vi "Build Message with Arguments++.vi"   [LabVIEW 2017, in "Communicable State Machine.lvlib"]
doc: "Builds CSM message strings and operation strings.\n\n\n> [!NOTE] <b>Message Building API</b>\n>\n> This type of API is only used to concatenate message strings and does not send messages directly. The strings need to be merged into the CSM state queue, and the messages will be sent and the operation executed within the Parse State Queue++ VI. If you are familiar with CSM rules, you do not need to use this type of API. You can type the corresponding message string or operation string directly into the string.\n\n\n> [!NOTE] <b>Polymorphic VI Options</b>\n> - Build Message with Arguments(Auto Check).vi: Concatenates message strings based on the input message symbols.\n> - Build Asynchronous Message with Arguments.vi: Concatenates and generates CSM asynchronous message strings. The message type symbol is `->`.\n> - Build No-Reply Asynchronous Message with Arguments.vi: Concatenates and generates CSM asynchronous message strings without reply. The message type symbol is `->|`.\n> - Build Synchronous Message with Arguments.vi: Concatenates and generates CSM synchronous message strings. The message type symbol is `-@`.\n> - Build Interrupt Broadcast Message.vi: Concatenates and generates CSM interrupt broadcast strings.\n> - Build Normal Broadcast Message.vi: Concatenates and generates CSM status broadcast strings.\n> - Build Register Message.vi: Concatenates and generates CSM register state operation strings.\n> - Build Unregister Message.vi: Concatenates and generates CSM unregister state operation strings.\n> - CSM - Replace Marks in Messages.vi: Replaces placeholders in message strings.\n> - CSM - Replace Mark with String Array.vi: Replaces tags in a single state string with strings from an array and merges them into a string describing a group of states.\n\n\n> [!NOTE] <b>CSM Inter-module Communication Types</b>\n>\n> Communication between CSM modules is divided into two categories: Messages and Broadcasts.\n> - <b>Messages</b>: 1:1 communication between modules. Based on the message handling method, it can be further divided into Synchronous Call (`-@`), Asynchronous Call (`->`), and Asynchronous Call without Reply (`->|`).\n> - <b>Broadcasts</b>: 1:N communication between modules. The broadcasting module pushes the broadcast to all modules registered to that broadcast. Based on the broadcast processing priority, it can be further divided into Status Broadcast and Interrupt Broadcast.\n\n\n### Build Message with Arguments(Auto Check).vi\nConcatenates and generates CSM message strings. The message type symbol is automatically detected based on the input <b>State with Arguments</b>.\n\n\n> [!NOTE] <b>Message Building API</b>\n>\n> This type of API is only used to concatenate message strings and does not send messages directly. The strings need to be merged into the CSM state queue, and the messages will be sent and the operation executed within the Parse State Queue++ VI. If you are familiar with CSM rules, you do not need to use this type of API. You can type the corresponding message string or operation string directly into the string.\n\n\n> [!NOTE] <b>CSM Message Target Module Description</b>\n>\n> In Normal Mode, the target module for a CSM message is the specified module name.\n> System-level modules start with a `.` in their name. The target module for a CSM message includes the `.` in the name. For example, if the requested module name is `.System`, the target module for the CSM message is `.System`.\n> In Worker Mode, the target module for a CSM message can only be the overall module name, not the node name. For example, if the requested module name is `Worker#`, the target module for the CSM message is `Worker`.\n> In Chain of Responsibility Mode, the target module for a CSM message can only be the overall module name, not the node name. For example, if the requested module name is `Chain$1`, the target module for the CSM message is `Chain`.\n\n\n-- <b>Controls</b> --\n- <b>State with Arguments</b>: CSM state string, which can contain arguments and target module information.\n- <b>Arguments (\"\")</b>: Argument information. Arguments contained in <b>State with Arguments</b> will be replaced.\n- <b>Target Module (\"\")</b>: Target module. If empty, the default module in <b>State with Arguments</b> will be used.\n\n-- <b>Indicators</b> --\n- <b>CSM Message String</b>: Concatenated CSM message string.\n\n### Build Synchronous Message with Arguments.vi\nConcatenates and generates CSM synchronous message strings. The message type symbol is `-@`, for example:\n\n Message >> Arguments -@ Target\n\n\n> [!NOTE] <b>Message Building API</b>\n>\n> This type of API is only used to concatenate message strings and does not send messages directly. The strings need to be merged into the CSM state queue, and the messages will be sent and the operation executed within the Parse State Queue++ VI. If you are familiar with CSM rules, you do not need to use this type of API. You can type the corresponding message string or operation string directly into the string.\n\n\n> [!NOTE] <b>Synchronous Message</b>\n>\n> A synchronous message is a type of message. After a CSM sends a synchronous message, it pauses state transitions and waits for the callee to complete message processing. Synchronous messages are described via `-@`. A call from one JKISM module to another via a synchronous message is called a synchronous call.\n>\n> <b>Errors occurring at the Caller</b>:\n> - If the input target module is `\"\"`, a `NO Target Error` is generated.\n> - If the input module does not exist, a `Target Error` is generated.\n> - If the input module exists but does not complete processing within the specified time, a `Timeout Error` is generated.\n>\n> <b>Caller waits for return</b>:\n> - If the caller is a CSM module, it stays in the Parse State the Queue++ VI.\n> - If it is an API call, it stays in the calling VI, such as the CSM - Send Message and Wait for Reply VI.\n>\n> <b>Return</b>:\n> - <b>If the caller is a CSM module</b>:\n> - Normally, it enters the `Response` state to handle the return.\n> - If an error occurs at the caller, it causes the CSM state machine to enter the `Error Handler` module to handle the error.\n> - If an error occurs at the callee, this information is still the result of the message. It is handled in the `Response` state and can be obtained from Additional Information.\n> - <b>If it is an API call</b>:\n> - The Response output is the return.\n> - Errors occurring at both the caller and callee are merged into the error cluster output.\n\n\n> [!NOTE] <b>CSM Message Target Module Description</b>\n>\n> In Normal Mode, the target module for a CSM message is the specified module name.\n> System-level modules start with a `.` in their name. The target module for a CSM message includes the `.` in the name. For example, if the requested module name is `.System`, the target module for the CSM message is `.System`.\n> In Worker Mode, the target module for a CSM message can only be the overall module name, not the node name. For example, if the requested module name is `Worker#`, the target module for the CSM message is `Worker`.\n> In Chain of Responsibility Mode, the target module for a CSM message can only be the overall module name, not the node name. For example, if the requested module name is `Chain$1`, the target module for the CSM message is `Chain`.\n\n\n-- <b>Controls</b> --\n- <b>State with Arguments</b>: CSM state string.\n- <b>Arguments (\"\")</b>: Argument information. Arguments contained in <b>State with Arguments</b> will be replaced.\n- <b>Target Module (\"\")</b>: Target module. If empty, the default module in <b>State with Arguments</b> will be used.\n\n-- <b>Indicators</b> --\n- <b>CSM Message String</b>: Concatenated CSM message string.\n\n### Build Asynchronous Message with Arguments.vi\nConcatenates and generates CSM asynchronous message strings. The message type symbol is `->`, for example:\n\n Message >> Arguments -> Target\n\n\n> [!NOTE] <b>Message Building API</b>\n>\n> This type of API is only used to concatenate message strings and does not send messages directly. The strings need to be merged into the CSM state queue, and the messages will be sent and the operation executed within the Parse State Queue++ VI. If you are familiar with CSM rules, you do not need to use this type of API. You can type the corresponding message string or operation string directly into the string.\n\n\n> [!NOTE] <b>Asynchronous Message</b>\n>\n> An asynchronous message is a type of message. After a CSM sends an asynchronous message, it immediately continues to execute subsequent code without waiting for the callee to complete message processing. Asynchronous messages are divided into Asynchronous Call (`->`) and Asynchronous Call without Reply (`->|`). The only difference is that with an Asynchronous Call without Reply (`->|`), the callee will not return the result to the caller after completing the operation.\n>\n> <b>Errors occurring at the Caller</b>:\n> - If the input target module is `\"\"`, a `NO Target Error` is generated.\n> - If the input module does not exist, a `Target Error` is generated.\n>\n> <b>Caller does not wait for return</b>:\n> - If the caller is a CSM module, it enters the `Async Message Posted` state after sending the message in the Parse State Queue++ VI.\n> - If it is an API call, it continues to execute subsequent code. The API can only send Asynchronous without Reply messages.\n>\n> <b>Return</b>:\n> - <b>If the caller is a CSM module</b>:\n> - Normally, it enters the `Async Response` state to handle the return. If an error occurs at the callee, this information is still the result of the message. It is handled in the `Async Response` state, and this error information can be obtained from Additional Information.\n> - If an error occurs at the caller, it causes the CSM state machine to enter the `Error Handler` module to handle the error.\n> - There is no return if the API can only send Asynchronous without Reply messages.\n\n\n> [!NOTE] <b>CSM Message Target Module Description</b>\n>\n> In Normal Mode, the target module for a CSM message is the specified module name.\n> System-level modules start with a `.` in their name. The target module for a CSM message includes the `.` in the name. For example, if the requested module name is `.System`, the target module for the CSM message is `.System`.\n> In Worker Mode, the target module for a CSM message can only be the overall module name, not the node name. For example, if the requested module name is `Worker#`, the target module for the CSM message is `Worker`.\n> In Chain of Responsibility Mode, the target module for a CSM message can only be the overall module name, not the node name. For example, if the requested module name is `Chain$1`, the target module for the CSM message is `Chain`.\n\n\n-- <b>Controls</b> --\n- <b>State with Arguments</b>: CSM state string.\n- <b>Arguments (\"\")</b>: Argument information. Arguments contained in <b>State with Arguments</b> will be replaced.\n- <b>Target Module (\"\")</b>: Target module. If empty, the default module in <b>State with Arguments</b> will be used.\n\n-- <b>Indicators</b> --\n- <b>CSM Message String</b>: Concatenated CSM message string.\n\n### Build No-Reply Asynchronous Message with Arguments.vi\nConcatenates and generates CSM asynchronous message strings without reply. The message type symbol is `->|`, for example:\n\n Message >> Arguments ->| Target\n\n\n> [!NOTE] <b>Message Building API</b>\n>\n> This type of API is only used to concatenate message strings and does not send messages directly. The strings need to be merged into the CSM state queue, and the messages will be sent and the operation executed within the Parse State Queue++ VI. If you are familiar with CSM rules, you do not need to use this type of API. You can type the corresponding message string or operation string directly into the string.\n\n\n> [!NOTE] <b>Asynchronous Message</b>\n>\n> An asynchronous message is a type of message. After a CSM sends an asynchronous message, it immediately continues to execute subsequent code without waiting for the callee to complete message processing. Asynchronous messages are divided into Asynchronous Call (`->`) and Asynchronous Call without Reply (`->|`). The only difference is that with an Asynchronous Call without Reply (`->|`), the callee will not return the result to the caller after completing the operation.\n>\n> <b>Errors occurring at the Caller</b>:\n> - If the input target module is `\"\"`, a `NO Target Error` is generated.\n> - If the input module does not exist, a `Target Error` is generated.\n>\n> <b>Caller does not wait for return</b>:\n> - If the caller is a CSM module, it enters the `Async Message Posted` state after sending the message in the Parse State Queue++ VI.\n> - If it is an API call, it continues to execute subsequent code. The API can only send Asynchronous without Reply messages.\n>\n> <b>Return</b>:\n> - <b>If the caller is a CSM module</b>:\n> - Normally, it enters the `Async Response` state to handle the return. If an error occurs at the callee, this information is still the result of the message. It is handled in the `Async Response` state, and this error information can be obtained from Additional Information.\n> - If an error occurs at the caller, it causes the CSM state machine to enter the `Error Handler` module to handle the error.\n> - There is no return if the API can only send Asynchronous without Reply messages.\n\n\n> [!NOTE] <b>CSM Message Target Module Description</b>\n>\n> In Normal Mode, the target module for a CSM message is the specified module name.\n> System-level modules start with a `.` in their name. The target module for a CSM message includes the `.` in the name. For example, if the requested module name is `.System`, the target module for the CSM message is `.System`.\n> In Worker Mode, the target module for a CSM message can only be the overall module name, not the node name. For example, if the requested module name is `Worker#`, the target module for the CSM message is `Worker`.\n> In Chain of Responsibility Mode, the target module for a CSM message can only be the overall module name, not the node name. For example, if the requested module name is `Chain$1`, the target module for the CSM message is `Chain`.\n\n\n-- <b>Controls</b> --\n- <b>State with Arguments</b>: CSM state string.\n- <b>Arguments (\"\")</b>: Argument information. Arguments contained in <b>State with Arguments</b> will be replaced.\n- <b>Target Module (\"\")</b>: Target module. If empty, the default module in <b>State with Arguments</b> will be used.\n\n-- <b>Indicators</b> --\n- <b>CSM Message String</b>: Concatenated CSM message string.\n\n### Build Status Broadcast Message.vi\nConcatenates normal status message strings. The message format is as follows:\n\n Status >> Arguments -><status>\n // The following strings are equivalent operations.\n // More operation characters are defined for easier typing and memorization.\n Status >> Arguments -><broadcast>\n Status >> Arguments -><all>\n\n\n> [!NOTE] <b>Message Building API</b>\n>\n> This type of API is only used to concatenate message strings and does not send messages directly. The strings need to be merged into the CSM state queue, and the messages will be sent and the operation executed within the Parse State Queue++ VI. If you are familiar with CSM rules, you do not need to use this type of API. You can type the corresponding message string or operation string directly into the string.\n\n\n-- <b>Controls</b> --\n- <b>State with Arguments</b>: CSM normal status message string.\n- <b>Arguments (\"\")</b>: Argument information. Arguments contained in <b>State with Arguments</b> will be replaced.\n\n-- <b>Indicators</b> --\n- <b>CSM Message String</b>: Concatenated CSM message string.\n\n### Build Interrupt Broadcast Message.vi\nConcatenates interrupt status messages. The message format is as follows:\n\n Status >> Arguments -><interrupt>\n\n\n> [!NOTE] <b>Message Building API</b>\n>\n> This type of API is only used to concatenate message strings and does not send messages directly. The strings need to be merged into the CSM state queue, and the messages will be sent and the operation executed within the Parse State Queue++ VI. If you are familiar with CSM rules, you do not need to use this type of API. You can type the corresponding message string or operation string directly into the string.\n\n\n-- <b>Controls</b> --\n- <b>State with Arguments</b>: CSM interrupt status message string.\n- <b>Arguments (\"\")</b>: Argument information. Arguments contained in <b>State with Arguments</b> will be replaced.\n\n-- <b>Indicators</b> --\n- <b>CSM Message String</b>: Concatenated CSM message string.\n\n### Build Register Message.vi\nConcatenates register state operation message strings. The message format is as follows:\n\n //[source-state]@[source-module] >> [response-message]@[response-module] -><register>\n status @ Source >> API @ Target -><register>\n\n Example: Bind the \"Download Finished\" message of the Downloader module to the \"Start Play\" API of the Player module.\n // Bind the \"Download Finished\" message of the Downloader module to the \"Start Play\" API of the Player module\n DownloadFinished@Downloader >> StartPlay@Player -><register>\n // When executing the message within the Player module, \"Player\" can be omitted\n DownloadFinished@Downloader >> StartPlay -><register>\n // When multiple modules have the \"Download Finished\" message,\n // use * to bind this message from all modules to the \"Start Play\" API of the Player module\n DownloadFinished@* >> StartPlay@Player -><register>\n\n\n> [!NOTE] <b>Message Building API</b>\n>\n> This type of API is only used to concatenate message strings and does not send messages directly. The strings need to be merged into the CSM state queue, and the messages will be sent and the operation executed within the Parse State Queue++ VI. If you are familiar with CSM rules, you do not need to use this type of API. You can type the corresponding message string or operation string directly into the string.\n\n\n> [!NOTE] <b>CSM Registration</b>\n>\n> Registration associates a broadcast with a bound interface (API). When the broadcast is triggered, the bound interface (API) is called. Registrations can also be cancelled. In CSM, there are two types of broadcasts:\n>\n> - <b>Broadcast</b>: Broadcast explicitly called by the module sending the broadcast message. Arguments need to be explicitly provided.\n> - <b>State</b>: Any state of a CSM module can also be registered to. The argument received by the triggered API is the Response of the CSM state.\n>\n> // Register\n> [CSM Broadcast]@[SourceModule] >> [Bound API]@[TargetModule] -><register> // [Comments]\n> // Unregister\n> [CSM Broadcast]@[SourceModule] >> [Bound API]@[TargetModule] -><unregister> // [Comments]\n>\n> - <b>CSM Broadcast</b>: Defined by the source module. Refer to \"CSM Broadcast Format Parsing\" for details.\n> - <b>Source Module</b>: The broadcasting module. If registering to broadcasts from any module, the source module can be represented by `*`.\n> - <b>Bound API</b>: Defined by the target module. It is the external interface of the target module.\n> - <b>Target Module</b>: The module where the bound API resides. When indicating registration to the current module within a CSM module, it can be ignored. The preceding `@` separator is also omitted.\n> - `<register>` / `<unregister>`: Definition of the Register/Unregister operation type.\n> - <b>Comments</b>: Comment information, which will not be parsed.\n\n\n> [!NOTE] <b>CSM Registration Location</b>\n>\n> There are two types of registration rules added by CSM registrations: Internal Addition and External Addition.\n> - <b>External Addition</b>: Rules added externally are global rules. They will not be automatically deleted when the CSM module exits and must be manually unregistered.\n> - Rules added using the `-<register>` statement are considered externally added if the module name where the API resides is specified.\n> - All rules added using the API CSM - Register Broadcast VI are considered externally added.\n> - <b>Internal Addition</b>: Rules added internally within a CSM module will be automatically deleted when the CSM module exits, so there is no need to manually unregister.\n> - Rules are considered internally added only when added using the `-<register>` statement and the API does not specify a module name.\n>\n> // Example:\n> status@sourceModule >> API@TargetModule -><register> // Externally added\n> status@sourceModule >> API -><register> // Internally added\n\n\n> [!NOTE] <b>CSM Broadcast Priority</b>\n>\n>Broadcasts have priorities. State broadcast is a special type of broadcast. By default, the priority of state broadcasts is the same as the priority of status broadcasts. Interrupt broadcasts are high-priority broadcasts and are passed using the high-priority queue, just like synchronous messages. Status broadcasts are low-priority broadcasts and are passed using the low-priority queue, just like asynchronous messages.\n>\n> // The default broadcast is a Status Broadcast, for example:\n> ModuleInternalChange >> Arguments -> <broadcast> // Low Priority\n> ModuleInternalChange >> Arguments -> <broadcast> // Low Priority\n>\n> The default priority is defined by the sender via the broadcast type in the broadcast format.\n>\n> // The sender can define the priority of the broadcast\n> ModuleInternalChange >> Arguments -> <status> // Low Priority\n> ModuleInternalChange >> Arguments -> <interrupt> // High Priority\n>\n> Default registrations do not change the priority, but the priority of the registered broadcast can be changed via special registration formats.\n>\n> // Default registration does not change priority\n> ModuleInternalChange@SourceModule >> API@TargetModule -><register>\n> // Change the registered broadcast to Normal priority, regardless of its original priority\n> ModuleInternalChange@SourceModule >> API@TargetModule -><register as status>\n> // Change the registered broadcast to High priority, regardless of its original priority\n> ModuleInternalChange@SourceModule >> API@TargetModule -><register as interrupt>\n\n\n-- <b>Controls</b> --\n- <b>Target CSM</b>: Name of the CSM module registering to the status.\n- <b>Source CSM (* as Default)</b>: Name of the CSM module publishing the status.\n- <b>Status</b>: Status to register.\n- <b>API (If \"\", Same As \"Status\")</b>: Name of the API in the registering module that responds to the status.\n- <b>Priority (No Change)</b>: Priority of the broadcast after registration.\n\n-- <b>Indicators</b> --\n- <b>CSM Message String</b>: Concatenated CSM message string.\n\n### Build Unregister Message.vi\nConcatenates unregister state operation message strings. The message format is as follows:\n\n //[source-state]@[source-module] >> [response-message]@[response-module] -><unregister>\n status @ Source >> API @ Target -><unregister>\n\n Example: Cancel the binding of the \"Download Finished\" message of the Downloader module to the \"Start Play\" API of the Player module.\n // Cancel binding of the \"Download Finished\" message of the Downloader module to the \"Start Play\" API of the Player module\n DownloadFinished@Downloader >> StartPlay@Player -><unregister>\n // When executing the message within the Player module, \"Player\" can be omitted\n DownloadFinished@Downloader >> StartPlay -><unregister>\n\n- In Worker Mode, the module's internal registration rules will only be automatically unregistered after all nodes have exited.\n- In Chain of Responsibility Mode, the module's internal registration rules will be automatically unregistered as the node exits.\n\n\n> [!NOTE] <b>Message Building API</b>\n>\n> This type of API is only used to concatenate message strings and does not send messages directly. The strings need to be merged into the CSM state queue, and the messages will be sent and the operation executed within the Parse State Queue++ VI. If you are familiar with CSM rules, you do not need to use this type of API. You can type the corresponding message string or operation string directly into the string.\n\n\n> [!NOTE] <b>CSM Registration</b>\n>\n> Registration associates a broadcast with a bound interface (API). When the broadcast is triggered, the bound interface (API) is called. Registrations can also be cancelled. In CSM, there are two types of broadcasts:\n>\n> - <b>Broadcast</b>: Broadcast explicitly called by the module sending the broadcast message. Arguments need to be explicitly provided.\n> - <b>State</b>: Any state of a CSM module can also be registered to. The argument received by the triggered API is the Response of the CSM state.\n>\n> // Register\n> [CSM Broadcast]@[SourceModule] >> [Bound API]@[TargetModule] -><register> // [Comments]\n> // Unregister\n> [CSM Broadcast]@[SourceModule] >> [Bound API]@[TargetModule] -><unregister> // [Comments]\n>\n> - <b>CSM Broadcast</b>: Defined by the source module. Refer to \"CSM Broadcast Format Parsing\" for details.\n> - <b>Source Module</b>: The broadcasting module. If registering to broadcasts from any module, the source module can be represented by `*`.\n> - <b>Bound API</b>: Defined by the target module. It is the external interface of the target module.\n> - <b>Target Module</b>: The module where the bound API resides. When indicating registration to the current module within a CSM module, it can be ignored. The preceding `@` separator is also omitted.\n> - `<register>` / `<unregister>`: Definition of the Register/Unregister operation type.\n> - <b>Comments</b>: Comment information, which will not be parsed.\n\n\n> [!NOTE] <b>CSM Registration Location</b>\n>\n> There are two types of registration rules added by CSM registrations: Internal Addition and External Addition.\n> - <b>External Addition</b>: Rules added externally are global rules. They will not be automatically deleted when the CSM module exits and must be manually unregistered.\n> - Rules added using the `-<register>` statement are considered externally added if the module name where the API resides is specified.\n> - All rules added using the API CSM - Register Broadcast VI are considered externally added.\n> - <b>Internal Addition</b>: Rules added internally within a CSM module will be automatically deleted when the CSM module exits, so there is no need to manually unregister.\n> - Rules are considered internally added only when added using the `-<register>` statement and the API does not specify a module name.\n>\n> // Example:\n> status@sourceModule >> API@TargetModule -><register> // Externally added\n> status@sourceModule >> API -><register> // Internally added\n\n\n-- <b>Controls</b> --\n- <b>Target CSM</b>: Name of the CSM module registering to the status.\n- <b>Source CSM (* as Default)</b>: Name of the CSM module publishing the status.\n- <b>Status</b>: Registered status.\n- <b>API (If \"\", Same As \"Status\")</b>: Name of the API in the registering module that responds to the status to be unregistered.\n\n-- <b>Indicators</b> --\n- <b>CSM Message String</b>: Concatenated CSM message string.\n\n### CSM - Replace Marks in Messages.vi\nFacilitates editing multiple CSM message strings by providing a batch replacement function for marks. There are four marks that can be replaced:\n- `<param>` mark: Usually represents the same argument.\n- `<target>` mark: Usually represents the same target.\n- `<1>` mark: Represents custom mark 1.\n- `<2>` mark: Represents custom mark 2.\n\n<b>Example</b>: The terminal `<target>` is connected to the string `DAQDevice`. The <b>States with Replace Token</b> string is:\n\n text\n Initialize -@ <target>\n Configure -@ <target>\n Read -@ <target>\n Close -@ <target>\n\nThe <b>States</b> output is:\n\n text\n Initialize -@ DAQDevice\n Configure -@ DAQDevice\n Read -@ DAQDevice\n Close -@ DAQDevice\n\n\n> [!NOTE] <b>Message Building API</b>\n>\n> This type of API is only used to concatenate message strings and does not send messages directly. The strings need to be merged into the CSM state queue, and the messages will be sent and the operation executed within the Parse State Queue++ VI. If you are familiar with CSM rules, you do not need to use this type of API. You can type the corresponding message string or operation string directly into the string.\n\n\n-- <b>Controls</b> --\n- <b>States with Replace Token</b>: CSM state string with replacement marks.\n- <b><param></b>: `<param>` mark, which usually represents the same argument.\n- <b><target></b>: `<target>` mark, which usually represents the same target.\n- <b><1></b>: Custom mark 1.\n- <b><2></b>: Custom mark 2.\n\n-- <b>Indicators</b> --\n- <b>States</b>: State string after replacement.\n\n### CSM - Replace Mark with String Array.vi\nReplaces tags in a single state string with strings from an array and merges them into a string describing a group of states.\n\n<b>Example</b>: For `Draw >> <1> -@ Painter`, <b>Tag</b> should be set to `<1>`\n\nInput array `[Line, Circle, Rectangle]`. The result will be:\n\n Draw >> Line -@ Painter\n Draw >> Circle -@ Painter\n Draw >> Rectangle -@ Painter\n\n-- <b>Controls</b> --\n- <b>single-line text</b>: Single-line state string containing tags like `<1>`, `<2>`, `<3>`, etc.\n- <b>Substitution Mark</b>: The tag to replace, such as `<1>`, `<2>`, `<3>`, etc.\n- <b>replace string</b>: The array of strings to replace the tag with.\n\n-- <b>Indicators</b> --\n- <b>States</b>: The merged state string."
uses:
  Communicable State Machine.lvlib
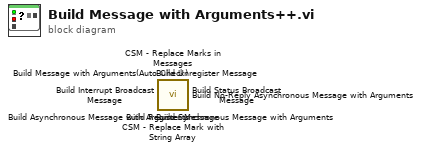
[diagram p0: block diagram]
diagram:
  n1 = call "Build Register Message.vi"() -> ()  [unwired: 15 in, 1 out]
  n2 = call "Build Unregister Message.vi"() -> ()  [unwired: 15 in, 1 out]
  n3 = call "Build Interrupt Broadcast Message.vi"() -> ()  [unwired: 15 in, 1 out]
  n4 = call "Build Status Broadcast Message.vi"() -> ()  [unwired: 15 in, 1 out]
  n5 = call "CSM - Replace Mark with String Array.vi"() -> ()  [unwired: 15 in, 1 out]
  n6 = call "CSM - Replace Marks in Messages.vi"() -> ()  [unwired: 15 in, 1 out]
  n7 = call "Build Message with Arguments(Auto Check).vi"() -> ()  [unwired: 15 in, 1 out]
  n8 = call "Build Synchronous Message with Arguments.vi"() -> ()  [unwired: 15 in, 1 out]
  n9 = call "Build No-Reply Asynchronous Message with Arguments.vi"() -> ()  [unwired: 15 in, 1 out]
  n10 = call "Build Asynchronous Message with Arguments.vi"() -> ()  [unwired: 15 in, 1 out]
